vi "VHistFile - Sorting time stamps.vi"(9 "time stamps in":dbl[](array[numeric]) format="%<%H:%M:%S%2u\n%d/%m/%Y>T") -> (0 "indexes out":i32[](array[numeric]), 1 "sorted":bool, 3 "time stamps out":dbl[](array[numeric]) format="%<%H:%M:%S%2u\n%d/%m/%Y>T")   [LabVIEW 2021]
doc: "::: CalcExpress Toolkit :::\nCopyright (c) 2000-2026 Konstantin Shifershteyn. All rights reserved."
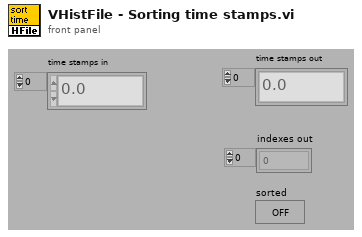
[diagram p1: front panel]
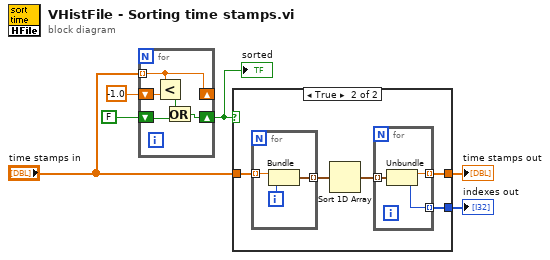
[diagram p0: block diagram]
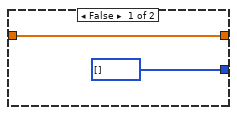
[diagram p2: hidden frame]
diagram:
  n1 = for {
    shift-right: [w8] -> _
    shift-left: -1.0 -> [w9]
    shift-right: [w10] -> w1
    shift-left: FALSE -> [w11]
    tunnel: "time stamps in" -> [w8] mode=indexing
    n2 = Less?(x=w8, y=w9) -> (x < y?=w7:bool)
    n3 = Or(x=w7, y=w11) -> (x .or. y?=w10:bool)
  }
  "sorted" <- w1
  n4 = case shown="True" w1 {
    tunnel: [i32[] [] w16] -> w6
    tunnel: [w13 w15] -> w5
    tunnel: "time stamps in" -> [w13 w14]
    frame False {
    }
    frame True {
      n5 = for {
        tunnel: w14 -> [w24] mode=indexing
        tunnel: [w22] -> w18 mode=indexing
        i -> [w23]
        n6 = Bundle("timestamp"=w24, w23) -> (w22:cluster{"timestamp":dbl, i32})  [unwired: 1 in]
      }
      n7 = Sort 1D Array(array=w18) -> (sorted array=w17:cluster{"timestamp":dbl, i32}[])
      n8 = for {
        tunnel: w17 -> [w21] mode=indexing
        tunnel: [w20] -> w16 mode=indexing
        tunnel: [w19] -> w15 mode=indexing
        n9 = Unbundle(w21) -> ("timestamp"=w19:dbl, w20:i32)
      }
    }
  }
  "time stamps out" <- w5
  "indexes out" <- w6
